vi "Kill Pin Map Service.vi"(8 "error in":errorcluster) -> (0 "error out":errorcluster)   [LabVIEW 2021, in "MeasurementServerTests.lvlib"]
uses:
  MeasurementServerTests.lvlib
  Runtime/Clients/Discovery V1/TypeDefs/gRPC Client Cache FGV Action.ctl
  Runtime/Clients/Discovery V1/NI Discovery V1 Client.lvlib
  Runtime/Clients/Pin Map V1/NI Pin Map V1 Client.lvlib
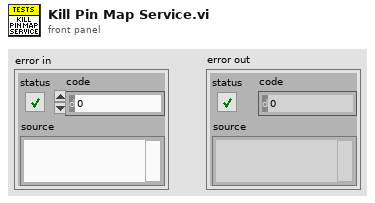
[diagram p1: front panel]
types:
  T1 = typedef "NI Discovery V1 Client.lvlib/gRPC Client Cache FGV Action.ctl" = enum16{"Get Client", "Recreate Client", "Destroy Client", "Update ClusterId"}
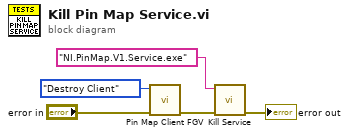
[diagram p0: block diagram]
diagram:
  n1 = call "Pin Map Client FGV.vi"("error in"="error in", "action"=gRPC_Client_Cache_FGV_Action."Destroy Client") -> ("error out"=w1:errorcluster)  [unwired: 7 in, 2 out]
  n2 = call "Kill Service.vi"("error in"=w1, "full exe name"="NI.PinMap.V1.Service.exe" ("command line")) -> ("error out"=→"error out":errorcluster)  [unwired: 9 in]
